vi "[ex ce] Zeroes and Extrema of f(x) .vi"() -> ()   [LabVIEW 2021]
doc: "CE-Math example.\n\n::: CalcExpress Toolkit :::\nCopyright (c) 2000-2026 Konstantin Shifershteyn. All rights reserved."
uses:
  <vilib>/gmath/NI_Gmath.lvlib
panel:
  in  "accuracy":dbl=1e-15
  in  "formula info":cluster{"formula":string, "x-variable":string}={"formula"="sinc(x)+sin(2*x)+sin(3*x)+sin(2*x**2)", "x-variable"="x"}
  in  "end":dbl=4.0 format="%.2f"
  in  "start":dbl format="%.2f"
  out "speed ratio":dbl format="%.3f"
  out "GM ticks":u32 caption="ms"
  out "CE ticks":u32 caption="ms"
  out "CE Graph":cluster{"x":dbl[], "f(x)":dbl[]}[](graph) caption="CalcExpress"
  in  "# points":u32=1000
  out "GM Graph":cluster{"x":dbl[], "f(x)":dbl[]}[](graph) caption="G Math"
  # "NOTE    CalcExpress uses (^) operator to perform bitwise-XOR operation but\nnot exponentiation operation. You have to use double-asterisk (**) operator\nto compute an exponent in a CalcExpress expression. For sample, x**y ."
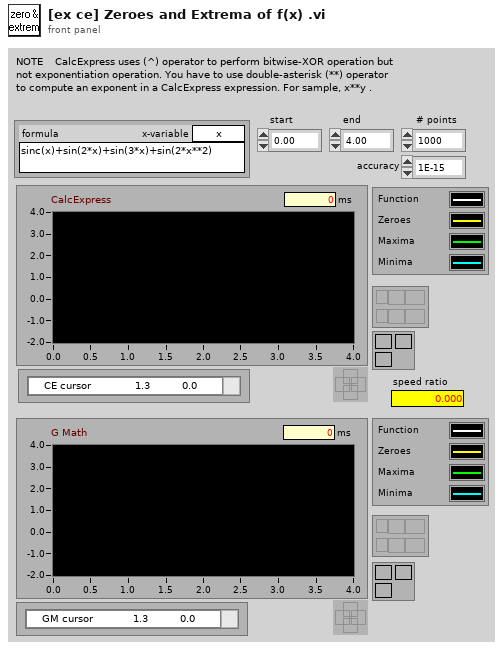
[diagram p1: front panel]
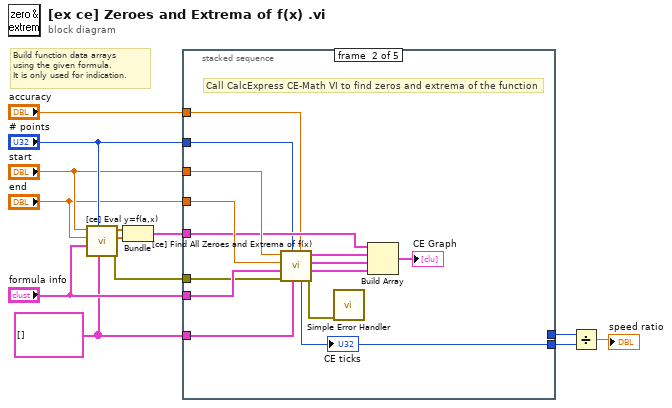
[diagram p0: block diagram]
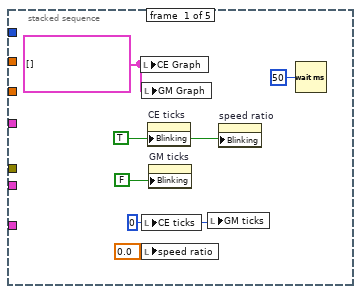
[diagram p2: hidden frame]
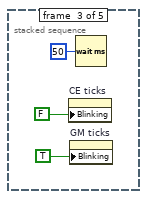
[diagram p3: hidden frame]
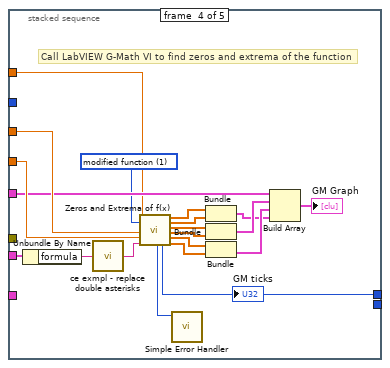
[diagram p4: hidden frame]
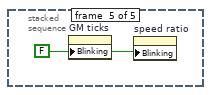
[diagram p5: hidden frame]
diagram:
  w2 = cluster{"name":string, "value":dbl}[] [] ("parameters")
  # "Build function data arrays\nusing the given formula.\nIt is only used for indication."
  n1 = call "[ce] Eval y=f(a,x).vi"("parameters"=w2, "# points"="# points", "formula info"="formula info", "end"="end", "start"="start") -> ("error out"=w3:errorcluster, "Y Values"=w5:dbl[], "X Values"=w6:dbl[])  [unwired: 3 in, 1 out]
  n2 = Bundle("X Values"=w6, "Y Values"=w5) -> (w4:cluster{"X Values":dbl[], "Y Values":dbl[]})  [unwired: 1 in]
  n3 = stacked-sequence {
    tunnel: "start" -> [_ w31 _ w53 _]
    tunnel: "end" -> [_ w30 _ w54 _]
    tunnel: "formula info" -> [_ w29 _ w52 _]
    tunnel: "# points" -> [_ w21 _ _ _]
    tunnel: [_ w32 _ _ _] -> w13
    tunnel: [_ _ _ w55 _] -> w11
    tunnel: w4 -> [_ w26 _ w42 _]
    tunnel: w3 -> [_ w23 _ _ _]
    tunnel: w2 -> [_ w22 _ _ _]
    tunnel: "accuracy" -> [_ w20 _ w40 _]
    frame #0 {
      w14 = cluster{"x":dbl[], "f(x)":dbl[]}[] [] ("CE Graph")
      w16 = u32 0 ("CE ticks")
      w18 = TRUE ("Write Attribute")
      n4 = local write "CE Graph"(w14) -> ()
      n5 = local write "GM Graph"(w14) -> ()
      n6 = local write "CE ticks"(w16) -> ()
      n7 = local write "speed ratio"(0.0 ("speed ratio")) -> ()
      n8 = property on="CE ticks" class="DigNum (strict)"("Blinking"=w18) -> ()  [unwired: 2 in, 2 out]
      n9 = property on="GM ticks" class="DigNum (strict)"("Blinking"=FALSE ("Write Attribute")) -> ()  [unwired: 2 in, 2 out]
      n10 = local write "GM ticks"(w16) -> ()
      n11 = property on="speed ratio" class="DigNum (strict)"("Blinking"=w18) -> ()  [unwired: 2 in, 2 out]
      n12 = Wait (ms)(milliseconds to wait=u32 50) -> ()  [unwired: 1 out]
    }
    frame #1 {
      # "Call CalcExpress CE-Math VI to find zeros and extrema of the function"
      n13 = call "[ce] Find All Zeroes and Extrema of f(x).vi"("accuracy"=w20, "parameters"=w22, "# points"=w21, "error in"=w23, "formula info"=w29, "end"=w30, "start"=w31) -> ("error out"=w33:errorcluster, "minima"=w27:cluster{"x":dbl[], "f(x)":dbl[]}, "maxima"=w24:cluster{"x":dbl[], "f(x)":dbl[]}, "zeroes"=w25:cluster{"x":dbl[], "f(x)":dbl[]}, "ticks"=w32:u32)
      "CE ticks" <- w32
      n14 = call <vilib>:"Simple Error Handler.vi"("error in (no error)"=w33) -> ()  [unwired: 4 in, 5 out]
      n15 = Build Array(w26, w25, w24, w27) -> (→"CE Graph":cluster{"x":dbl[], "f(x)":dbl[]}[])
    }
    frame #2 {
      n16 = property on="CE ticks" class="DigNum (strict)"("Blinking"=FALSE ("Write Attribute")) -> ()  [unwired: 2 in, 2 out]
      n17 = property on="GM ticks" class="DigNum (strict)"("Blinking"=TRUE ("Write Attribute")) -> ()  [unwired: 2 in, 2 out]
      n18 = Wait (ms)(milliseconds to wait=u32 50) -> ()  [unwired: 1 out]
    }
    frame #3 {
      w39 = u16 1 items=["fixed function", "modified function"] ("step type")
      # "Call LabVIEW G-Math VI to find zeros and extrema of the function"
      n19 = Unbundle By Name(w52) -> ("formula"=w38:string)
      n20 = call "ce exmpl - replace double asterisks .vi"("formula in"=w38) -> ("formula out"=w37:string)  [unwired: 4 in]
      n21 = call <vilib>:"Zeros and Extrema of f(x).vi"("accuracy"=w40, "step type"=w39, "start"=w53, "end"=w54, "formula"=w37) -> ("error"=w56:i32, "ticks"=w55:u32, "Minima"=w49:dbl[], "f(Minima)"=w48:dbl[], "Zeros"=w51:dbl[], "f(Zeros)"=w50:dbl[], "Maxima"=w47:dbl[], "f(Maxima)"=w46:dbl[])  [unwired: 7 in]
      "GM ticks" <- w55
      n22 = call <vilib>:"Simple Error Handler.vi"("error code (no error:0)"=w56) -> ()  [unwired: 4 in, 5 out]
      n23 = Bundle("Minima"=w49, "f(Minima)"=w48) -> (w43:cluster{"Minima":dbl[], "f(Minima)":dbl[]})  [unwired: 1 in]
      n24 = Bundle("Zeros"=w51, "f(Zeros)"=w50) -> (w45:cluster{"Zeros":dbl[], "f(Zeros)":dbl[]})  [unwired: 1 in]
      n25 = Bundle("Maxima"=w47, "f(Maxima)"=w46) -> (w44:cluster{"Maxima":dbl[], "f(Maxima)":dbl[]})  [unwired: 1 in]
      n26 = Build Array(w42, w45, w44, w43) -> (→"GM Graph":cluster{"Minima":dbl[], "f(Minima)":dbl[]}[])
    }
    frame #4 {
      w57 = FALSE ("Write Attribute")
      n27 = property on="GM ticks" class="DigNum (strict)"("Blinking"=w57) -> ()  [unwired: 2 in, 2 out]
      n28 = property on="speed ratio" class="DigNum (strict)"("Blinking"=w57) -> ()  [unwired: 2 in, 2 out]
    }
  }
  n29 = Divide(x=w11, y=w13) -> (x/y=→"speed ratio":dbl)
